vi "read_subtable_key_string.vi"(7 "subtables":string[](array[string]), 8 "error in (no error)":errorcluster, 9 "default (\"\")":string, 10 "subkeys":string[](array[string]), 11 "toml in":refnum<class "toml.lvclass">) -> (0 "error out":errorcluster, 1 "value":string="6.6.6", 2 "found?":bool, 3 "toml out":refnum<class "toml.lvclass">)   [LabVIEW 2020, in "toml.lvclass"]
uses:
  toml.lvclass
  toml.lvclass/toml.ctl
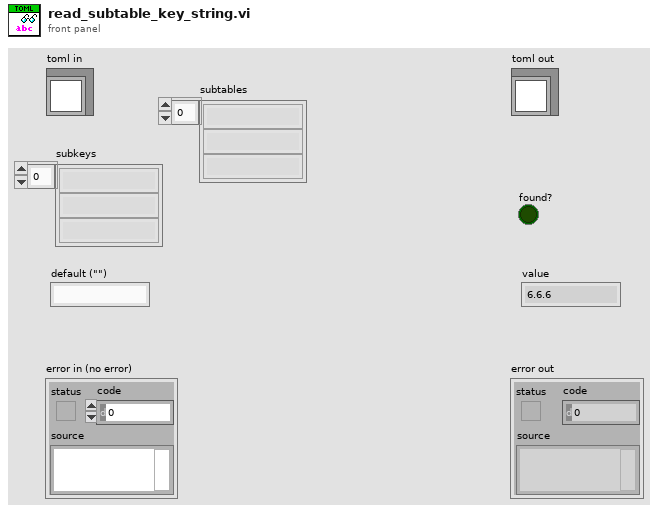
[diagram p1: front panel]
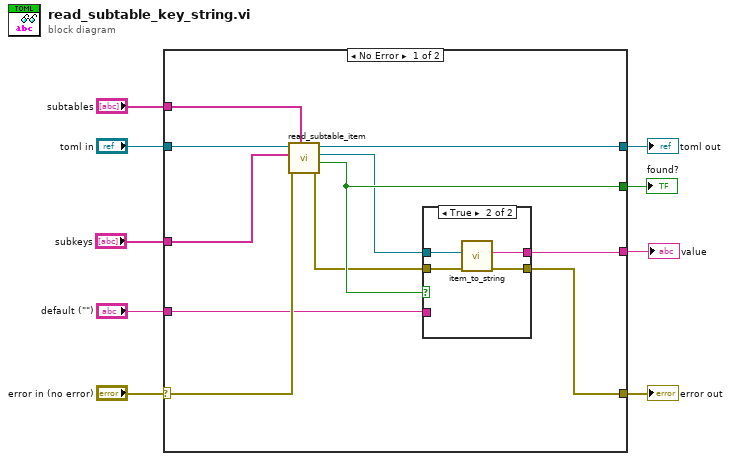
[diagram p0: block diagram]
diagram:
  n1 = case shown="No Error" "error in (no error)" {
    selector: "error in (no error)" -> [w18 w28]
    tunnel: [w13 w28] -> w8
    tunnel: [w19 w27] -> w6
    tunnel: "toml in" -> [w20 w27]
    tunnel: "subtables" -> [w11 _]
    tunnel: "subkeys" -> [w10 _]
    tunnel: "default (\"\")" -> [w14 _]
    tunnel: [w12 _] -> w2
    tunnel: [w17 _] -> w1
    frame No Error {
      n2 = call "read_subtable_item.vi"("subtables"=w11, "error in (no error)"=w18, "subkeys"=w10, "toml in"=w20) -> ("error out"=w16:errorcluster, "found?"=w17:bool, "item (value)"=w15:refnum<class "Item.lvclass">, "toml out"=w19:refnum<class "toml.lvclass">)  [unwired: 4 in]
      n3 = case shown="True" w17 {
        tunnel: w16 -> [w22 w26]
        tunnel: [w22 w25] -> w13
        tunnel: w15 -> [_ w24]
        tunnel: [w21 w23] -> w12
        tunnel: w14 -> [w21 _]
        frame False {
        }
        frame True {
          n4 = call "item_to_string.vi"("error in (no error)"=w26, "Item in"=w24) -> ("error out"=w25:errorcluster, "string_value"=w23:string)  [unwired: 8 in]
        }
      }
    }
    frame Error {
    }
  }
  "error out" <- w8
  "toml out" <- w6
  "value" <- w2
  "found?" <- w1
